vi "XY8_Pulse_Manipulation.vi"(8 "Numeric 2":i32, 9 "Invert?":bool, 10 "Numeric":i32, 11 "MW Step Size":dbl=2e-09) -> (3 "Tau":dbl)   [LabVIEW 2024]
uses:
  <vilib>/Utility/error.llb/DialogTypeEnum.ctl
  SpinCore_API_file_location.vi
panel:
  out "output array 2":T1(array[cluster])
  in  "clock_freq (MHz) 2":dbl=500.0
  out "x+y 11":dbl
  out "x+y 10":dbl
  out "x+y 9":dbl
  out "x+y 8":dbl
  out "x+y 7":dbl
  out "x+y 39":dbl
  out "x+y 38":dbl
  out "x+y 37":dbl
  out "x+y 36":dbl
  out "x+y 35":dbl
  out "x+y 34":dbl
  out "x+y 33":dbl
  out "x+y 32":dbl
  out "x+y 31":dbl
  out "x+y 30":dbl
  out "x+y 29":dbl
  out "x+y 28":dbl
  out "x+y 27":dbl
  out "x+y 26":dbl
  out "x+y 25":dbl
  out "x+y 24":dbl
  out "x+y 23":dbl
  out "x+y 22":dbl
  out "x+y 21":dbl
  out "x+y 20":dbl
  out "x+y 19":dbl
  out "x+y 18":dbl
  out "x+y 17":dbl
  out "x+y 16":dbl
  out "x+y 15":dbl
  out "x+y 14":dbl
  out "x+y 13":dbl
  out "x+y 12":dbl
  in  "# of Instructions":u32=49
  in  "Instructions":T1(array[cluster])=[{"Instruct Data"=0, "Op Code"=0, "Flags"=[FALSE, FALSE, TRUE, FALSE, FALSE, FALSE, FALSE, TRUE, FALSE, FALSE, FALSE, FALSE, FALSE, FALSE, FALSE, FALSE, FALSE, FALSE, FALSE, FALSE, FALSE, FALSE, FALSE, TRUE], "Comments"="0 Triggers", "Time (s)"=1e-07}, {"Instruct Data"=0, "Op Code"=0, "Flags"=[FALSE, FALSE, FALSE, FALSE, FALSE, FALSE, FALSE, TRUE, FALSE, FALSE, FALSE, FALSE, FALSE, FALSE, FALSE, FALSE, FALSE, FALSE, FALSE, FALSE, FALSE, FALSE, FALSE, FALSE], "Comments"="1 Dark ", "Time (s)"=0.00024}, {"Instruct Data"=0, "Op Code"=0, "Flags"=[FALSE, FALSE, FALSE, FALSE, FALSE, FALSE, FALSE, TRUE, FALSE, FALSE, FALSE, FALSE, FALSE, FALSE, FALSE, FALSE, FALSE, FALSE, FALSE, FALSE, FALSE, FALSE, FALSE, FALSE], "Comments"="2 AOM Buffer", "Time (s)"=5e-07}, {"Instruct Data"=0, "Op Code"=0, "Flags"=[TRUE, FALSE, FALSE, TRUE, FALSE, FALSE, FALSE, TRUE, FALSE, FALSE, FALSE, FALSE, FALSE, FALSE, FALSE, FALSE, FALSE, FALSE, FALSE, FALSE, FALSE, FALSE, FALSE, FALSE], "Comments"="3 pi/2", "Time (s)"=3.6e-08}, {"Instruct Data"=0, "Op Code"=0, "Flags"=[FALSE, FALSE, FALSE, FALSE, FALSE, FALSE, FALSE, TRUE, FALSE, FALSE, FALSE, FALSE, FALSE, FALSE, FALSE, FALSE, FALSE, FALSE, FALSE, FALSE, FALSE, FALSE, FALSE, FALSE], "Comments"="4 tau/2", "Time (s)"=2.313e-05}, {"Instruct Data"=0, "Op Code"=0, "Flags"=[TRUE, FALSE, FALSE, TRUE, FALSE, FALSE, FALSE, TRUE, FALSE, FALSE, FALSE, FALSE, FALSE, FALSE, FALSE, FALSE, FALSE, FALSE, FALSE, FALSE, FALSE, FALSE, FALSE, FALSE], "Comments"="5  Pi_X", "Time (s)"=6.7e-08}, {"Instruct Data"=0, "Op Code"=0, "Flags"=[FALSE, FALSE, FALSE, FALSE, FALSE, FALSE, FALSE, TRUE, FALSE, FALSE, FALSE, FALSE, FALSE, FALSE, FALSE, FALSE, FALSE, FALSE, FALSE, FALSE, FALSE, FALSE, FALSE, FALSE], "Comments"="6 Tau", "Time (s)"=4.626e-05}, {"Instruct Data"=0, "Op Code"=0, "Flags"=[TRUE, FALSE, FALSE, FALSE, TRUE, FALSE, FALSE, TRUE, FALSE, FALSE, FALSE, FALSE, FALSE, FALSE, FALSE, FALSE, FALSE, FALSE, FALSE, FALSE, FALSE, FALSE, FALSE, FALSE], "Comments"="7 Pi_Y", "Time (s)"=7e-08}, {"Instruct Data"=0, "Op Code"=0, "Flags"=[FALSE, FALSE, FALSE, FALSE, FALSE, FALSE, FALSE, TRUE, FALSE, FALSE, FALSE, FALSE, FALSE, FALSE, FALSE, FALSE, FALSE, FALSE, FALSE, FALSE, FALSE, FALSE, FALSE, FALSE], "Comments"="8 Tau", "Time (s)"=4.626e-05}, {"Instruct Data"=0, "Op Code"=0, "Flags"=[TRUE, FALSE, FALSE, TRUE, FALSE, FALSE, FALSE, TRUE, FALSE, FALSE, FALSE, FALSE, FALSE, FALSE, FALSE, FALSE, FALSE, FALSE, FALSE, FALSE, FALSE, FALSE, FALSE, FALSE], "Comments"="9 Pi_X", "Time (s)"=6.7e-08}, {"Instruct Data"=0, "Op Code"=0, "Flags"=[FALSE, FALSE, FALSE, FALSE, FALSE, FALSE, FALSE, TRUE, FALSE, FALSE, FALSE, FALSE, FALSE, FALSE, FALSE, FALSE, FALSE, FALSE, FALSE, FALSE, FALSE, FALSE, FALSE, FALSE], "Comments"="10 tau", "Time (s)"=4.626e-05}, {"Instruct Data"=0, "Op Code"=0, "Flags"=[TRUE, FALSE, FALSE, FALSE, TRUE, FALSE, FALSE, TRUE, FALSE, FALSE, FALSE, FALSE, FALSE, FALSE, FALSE, FALSE, FALSE, FALSE, FALSE, FALSE, FALSE, FALSE, FALSE, FALSE], "Comments"="11 Pi_Y", "Time (s)"=7e-08}, {"Instruct Data"=0, "Op Code"=0, "Flags"=[FALSE, FALSE, FALSE, FALSE, FALSE, FALSE, FALSE, TRUE, FALSE, FALSE, FALSE, FALSE, FALSE, FALSE, FALSE, FALSE, FALSE, FALSE, FALSE, FALSE, FALSE, FALSE, FALSE, FALSE], "Comments"="12 Tau", "Time (s)"=4.626e-05}, {"Instruct Data"=0, "Op Code"=0, "Flags"=[TRUE, FALSE, FALSE, FALSE, TRUE, FALSE, FALSE, TRUE, FALSE, FALSE, FALSE, FALSE, FALSE, FALSE, FALSE, FALSE, FALSE, FALSE, FALSE, FALSE, FALSE, FALSE, FALSE, FALSE], "Comments"="13 Pi_Y", "Time (s)"=7e-08}, {"Instruct Data"=0, "Op Code"=0, "Flags"=[FALSE, FALSE, FALSE, FALSE, FALSE, FALSE, FALSE, TRUE, FALSE, FALSE, FALSE, FALSE, FALSE, FALSE, FALSE, FALSE, FALSE, FALSE, FALSE, FALSE, FALSE, FALSE, FALSE, FALSE], "Comments"="14 tau", "Time (s)"=4.626e-05}, {"Instruct Data"=0, "Op Code"=0, "Flags"=[TRUE, FALSE, FALSE, TRUE, FALSE, FALSE, FALSE, TRUE, FALSE, FALSE, FALSE, FALSE, FALSE, FALSE, FALSE, FALSE, FALSE, FALSE, FALSE, FALSE, FALSE, FALSE, FALSE, FALSE], "Comments"="15 Pi_X", "Time (s)"=6.7e-08}, {"Instruct Data"=0, "Op Code"=0, "Flags"=[FALSE, FALSE, FALSE, FALSE, FALSE, FALSE, FALSE, TRUE, FALSE, FALSE, FALSE, FALSE, FALSE, FALSE, FALSE, FALSE, FALSE, FALSE, FALSE, FALSE, FALSE, FALSE, FALSE, FALSE], "Comments"="16  tau", "Time (s)"=4.626e-05}, {"Instruct Data"=0, "Op Code"=0, "Flags"=[TRUE, FALSE, FALSE, FALSE, TRUE, FALSE, FALSE, TRUE, FALSE, FALSE, FALSE, FALSE, FALSE, FALSE, FALSE, FALSE, FALSE, FALSE, FALSE, FALSE, FALSE, FALSE, FALSE, FALSE], "Comments"="17 Pi_Y", "Time (s)"=7e-08}, {"Instruct Data"=0, "Op Code"=0, "Flags"=[FALSE, FALSE, FALSE, FALSE, FALSE, FALSE, FALSE, TRUE, FALSE, FALSE, FALSE, FALSE, FALSE, FALSE, FALSE, FALSE, FALSE, FALSE, FALSE, FALSE, FALSE, FALSE, FALSE, FALSE], "Comments"="18 tau", "Time (s)"=4.626e-05}, {"Instruct Data"=0, "Op Code"=0, "Flags"=[TRUE, FALSE, FALSE, TRUE, FALSE, FALSE, FALSE, TRUE, FALSE, FALSE, FALSE, FALSE, FALSE, FALSE, FALSE, FALSE, FALSE, FALSE, FALSE, FALSE, FALSE, FALSE, FALSE, FALSE], "Comments"="19 pi_X", "Time (s)"=6.7e-08}, {"Instruct Data"=0, "Op Code"=0, "Flags"=[FALSE, FALSE, FALSE, FALSE, FALSE, FALSE, FALSE, TRUE, FALSE, FALSE, FALSE, FALSE, FALSE, FALSE, FALSE, FALSE, FALSE, FALSE, FALSE, FALSE, FALSE, FALSE, FALSE, FALSE], "Comments"="20  tau/2", "Time (s)"=2.313e-05}, {"Instruct Data"=0, "Op Code"=0, "Flags"=[TRUE, FALSE, FALSE, TRUE, FALSE, FALSE, FALSE, TRUE, FALSE, FALSE, FALSE, FALSE, FALSE, FALSE, FALSE, FALSE, FALSE, FALSE, FALSE, FALSE, FALSE, FALSE, FALSE, FALSE], "Comments"="21 pi/2", "Time (s)"=3.6e-08}, {"Instruct Data"=0, "Op Code"=0, "Flags"=[FALSE, TRUE, FALSE, FALSE, FALSE, FALSE, FALSE, TRUE, FALSE, FALSE, FALSE, FALSE, FALSE, FALSE, FALSE, FALSE, FALSE, FALSE, FALSE, FALSE, FALSE, FALSE, FALSE, FALSE], "Comments"="22 AOM Buffer", "Time (s)"=5e-07}, {"Instruct Data"=0, "Op Code"=0, "Flags"=[FALSE, TRUE, FALSE, FALSE, FALSE, FALSE, FALSE, FALSE, FALSE, FALSE, FALSE, FALSE, FALSE, FALSE, FALSE, FALSE, FALSE, FALSE, FALSE, FALSE, FALSE, FALSE, FALSE, FALSE], "Comments"="23  Inhibit off", "Time (s)"=5e-07}, {"Instruct Data"=0, "Op Code"=0, "Flags"=[FALSE, TRUE, FALSE, FALSE, FALSE, FALSE, FALSE, TRUE, FALSE, FALSE, FALSE, FALSE, FALSE, FALSE, FALSE, FALSE, FALSE, FALSE, FALSE, FALSE, FALSE, FALSE, FALSE, FALSE], "Comments"="24  AOM", "Time (s)"=5e-06}, {"Instruct Data"=0, "Op Code"=0, "Flags"=[FALSE, FALSE, FALSE, FALSE, FALSE, FALSE, FALSE, TRUE, FALSE, FALSE, FALSE, FALSE, FALSE, FALSE, FALSE, FALSE, FALSE, FALSE, FALSE, FALSE, FALSE, FALSE, FALSE, FALSE], "Comments"="25  Dark", "Time (s)"=0.00024}, {"Instruct Data"=0, "Op Code"=0, "Flags"=[FALSE, FALSE, FALSE, FALSE, FALSE, FALSE, FALSE, TRUE, FALSE, FALSE, FALSE, FALSE, FALSE, FALSE, FALSE, FALSE, FALSE, FALSE, FALSE, FALSE, FALSE, FALSE, FALSE, FALSE], "Comments"="26  AOm buffer", "Time (s)"=5e-07}, {"Instruct Data"=0, "Op Code"=0, "Flags"=[TRUE, FALSE, FALSE, TRUE, FALSE, FALSE, FALSE, TRUE, FALSE, FALSE, FALSE, FALSE, FALSE, FALSE, FALSE, FALSE, FALSE, FALSE, FALSE, FALSE, FALSE, FALSE, FALSE, FALSE], "Comments"="27  pi/2", "Time (s)"=3.6e-08}, {"Instruct Data"=0, "Op Code"=0, "Flags"=[FALSE, FALSE, FALSE, FALSE, FALSE, FALSE, FALSE, TRUE, FALSE, FALSE, FALSE, FALSE, FALSE, FALSE, FALSE, FALSE, FALSE, FALSE, FALSE, FALSE, FALSE, FALSE, FALSE, FALSE], "Comments"="28  tau/2", "Time (s)"=2.313e-05}, {"Instruct Data"=0, "Op Code"=0, "Flags"=[TRUE, FALSE, FALSE, TRUE, FALSE, FALSE, FALSE, TRUE, FALSE, FALSE, FALSE, FALSE, FALSE, FALSE, FALSE, FALSE, FALSE, FALSE, FALSE, FALSE, FALSE, FALSE, FALSE, FALSE], "Comments"="29  pi_X", "Time (s)"=6.7e-08}, {"Instruct Data"=0, "Op Code"=0, "Flags"=[FALSE, FALSE, FALSE, FALSE, FALSE, FALSE, FALSE, TRUE, FALSE, FALSE, FALSE, FALSE, FALSE, FALSE, FALSE, FALSE, FALSE, FALSE, FALSE, FALSE, FALSE, FALSE, FALSE, FALSE], "Comments"="30  tau", "Time (s)"=4.626e-05}, {"Instruct Data"=0, "Op Code"=0, "Flags"=[TRUE, FALSE, FALSE, FALSE, TRUE, FALSE, FALSE, TRUE, FALSE, FALSE, FALSE, FALSE, FALSE, FALSE, FALSE, FALSE, FALSE, FALSE, FALSE, FALSE, FALSE, FALSE, FALSE, FALSE], "Comments"="31  Pi_y", "Time (s)"=7e-08}, {"Instruct Data"=0, "Op Code"=0, "Flags"=[FALSE, FALSE, FALSE, FALSE, FALSE, FALSE, FALSE, TRUE, FALSE, FALSE, FALSE, FALSE, FALSE, FALSE, FALSE, FALSE, FALSE, FALSE, FALSE, FALSE, FALSE, FALSE, FALSE, FALSE], "Comments"="32  tau", "Time (s)"=4.626e-05}, {"Instruct Data"=0, "Op Code"=0, "Flags"=[TRUE, FALSE, FALSE, TRUE, FALSE, FALSE, FALSE, TRUE, FALSE, FALSE, FALSE, FALSE, FALSE, FALSE, FALSE, FALSE, FALSE, FALSE, FALSE, FALSE, FALSE, FALSE, FALSE, FALSE], "Comments"="33  Pi_X", "Time (s)"=6.7e-08}, {"Instruct Data"=0, "Op Code"=0, "Flags"=[FALSE, FALSE, FALSE, FALSE, FALSE, FALSE, FALSE, TRUE, FALSE, FALSE, FALSE, FALSE, FALSE, FALSE, FALSE, FALSE, FALSE, FALSE, FALSE, FALSE, FALSE, FALSE, FALSE, FALSE], "Comments"="34  tau", "Time (s)"=4.626e-05}, {"Instruct Data"=0, "Op Code"=0, "Flags"=[TRUE, FALSE, FALSE, FALSE, TRUE, FALSE, FALSE, TRUE, FALSE, FALSE, FALSE, FALSE, FALSE, FALSE, FALSE, FALSE, FALSE, FALSE, FALSE, FALSE, FALSE, FALSE, FALSE, FALSE], "Comments"="35 Pi_Y", "Time (s)"=7e-08}, {"Instruct Data"=0, "Op Code"=0, "Flags"=[FALSE, FALSE, FALSE, FALSE, FALSE, FALSE, FALSE, TRUE, FALSE, FALSE, FALSE, FALSE, FALSE, FALSE, FALSE, FALSE, FALSE, FALSE, FALSE, FALSE, FALSE, FALSE, FALSE, FALSE], "Comments"="36  tau", "Time (s)"=4.626e-05}, {"Instruct Data"=0, "Op Code"=0, "Flags"=[TRUE, FALSE, FALSE, FALSE, TRUE, FALSE, FALSE, TRUE, FALSE, FALSE, FALSE, FALSE, FALSE, FALSE, FALSE, FALSE, FALSE, FALSE, FALSE, FALSE, FALSE, FALSE, FALSE, FALSE], "Comments"="37  Pi_Y", "Time (s)"=7e-08}, {"Instruct Data"=0, "Op Code"=0, "Flags"=[FALSE, FALSE, FALSE, FALSE, FALSE, FALSE, FALSE, TRUE, FALSE, FALSE, FALSE, FALSE, FALSE, FALSE, FALSE, FALSE, FALSE, FALSE, FALSE, FALSE, FALSE, FALSE, FALSE, FALSE], "Comments"="38  tau", "Time (s)"=4.626e-05}, {"Instruct Data"=0, "Op Code"=0, "Flags"=[TRUE, FALSE, FALSE, TRUE, FALSE, FALSE, FALSE, TRUE, FALSE, FALSE, FALSE, FALSE, FALSE, FALSE, FALSE, FALSE, FALSE, FALSE, FALSE, FALSE, FALSE, FALSE, FALSE, FALSE], "Comments"="39  Pi_X", "Time (s)"=6.7e-08}, {"Instruct Data"=0, "Op Code"=0, "Flags"=[FALSE, FALSE, FALSE, FALSE, FALSE, FALSE, FALSE, TRUE, FALSE, FALSE, FALSE, FALSE, FALSE, FALSE, FALSE, FALSE, FALSE, FALSE, FALSE, FALSE, FALSE, FALSE, FALSE, FALSE], "Comments"="40  tau", "Time (s)"=4.626e-05}, {"Instruct Data"=0, "Op Code"=0, "Flags"=[TRUE, FALSE, FALSE, FALSE, TRUE, FALSE, FALSE, TRUE, FALSE, FALSE, FALSE, FALSE, FALSE, FALSE, FALSE, FALSE, FALSE, FALSE, FALSE, FALSE, FALSE, FALSE, FALSE, FALSE], "Comments"="41  pi_Y", "Time (s)"=7e-08}, {"Instruct Data"=0, "Op Code"=0, "Flags"=[FALSE, FALSE, FALSE, FALSE, FALSE, FALSE, FALSE, TRUE, FALSE, FALSE, FALSE, FALSE, FALSE, FALSE, FALSE, FALSE, FALSE, FALSE, FALSE, FALSE, FALSE, FALSE, FALSE, FALSE], "Comments"="42  tau", "Time (s)"=4.626e-05}, {"Instruct Data"=0, "Op Code"=0, "Flags"=[TRUE, FALSE, FALSE, TRUE, FALSE, FALSE, FALSE, TRUE, FALSE, FALSE, FALSE, FALSE, FALSE, FALSE, FALSE, FALSE, FALSE, FALSE, FALSE, FALSE, FALSE, FALSE, FALSE, FALSE], "Comments"="43  Pi_x", "Time (s)"=6.7e-08}, {"Instruct Data"=0, "Op Code"=0, "Flags"=[FALSE, FALSE, FALSE, FALSE, FALSE, FALSE, FALSE, TRUE, FALSE, FALSE, FALSE, FALSE, FALSE, FALSE, FALSE, FALSE, FALSE, FALSE, FALSE, FALSE, FALSE, FALSE, FALSE, FALSE], "Comments"="44  tau/2", "Time (s)"=2.313e-05}, {"Instruct Data"=0, "Op Code"=0, "Flags"=[TRUE, FALSE, FALSE, TRUE, FALSE, FALSE, FALSE, TRUE, FALSE, FALSE, FALSE, FALSE, FALSE, FALSE, FALSE, FALSE, FALSE, FALSE, FALSE, FALSE, FALSE, FALSE, FALSE, FALSE], "Comments"="45  3Pi/2", "Time (s)"=1.01e-07}, {"Instruct Data"=0, "Op Code"=0, "Flags"=[FALSE, TRUE, FALSE, FALSE, FALSE, FALSE, FALSE, TRUE, FALSE, FALSE, FALSE, FALSE, FALSE, FALSE, FALSE, FALSE, FALSE, FALSE, FALSE, FALSE, FALSE, FALSE, FALSE, FALSE], "Comments"="46  AOM Buffer", "Time (s)"=5e-07}, {"Instruct Data"=0, "Op Code"=0, "Flags"=[FALSE, TRUE, FALSE, FALSE, FALSE, FALSE, FALSE, FALSE, FALSE, FALSE, FALSE, FALSE, FALSE, FALSE, FALSE, FALSE, FALSE, FALSE, FALSE, FALSE, FALSE, FALSE, FALSE, FALSE], "Comments"="47  Inhibit off", "Time (s)"=5e-07}, {"Instruct Data"=0, "Op Code"=6, "Flags"=[FALSE, TRUE, FALSE, FALSE, FALSE, FALSE, FALSE, TRUE, FALSE, FALSE, FALSE, FALSE, FALSE, FALSE, FALSE, FALSE, FALSE, FALSE, FALSE, FALSE, FALSE, FALSE, FALSE, FALSE], "Comments"="48  AOM", "Time (s)"=5e-06}] {"Time (s)" format="%.3p"; "Op Code" items=["Continue", "Stop", "Loop", "End Loop", "JSR", "RTS", "Branch", "Long Delay", "Wait"]}
  out "output array":T1(array[cluster])
  in  "clock_freq (MHz)":dbl=500.0
  out "x+y 2":dbl
  out "x+y 3":dbl
  out "x+y 4":dbl
  out "x+y 5":dbl
  out "x+y 6":dbl
  # "1"
  # "2"
  # "3"
  # "4"
  # "5"
  # "6"
  # "7"
  # "8"
  # "9"
  # "10"
  # "11"
  # "12"
  # "13"
  # "14"
  # "15"
  # "16"
  # "17"
  # "18"
  # "19"
  # "20"
  # "21"
  # "22"
  # "23"
  # "24"
types:
  T1 = cluster{"Instruct Data":i32, "Op Code":i32, "Flags":bool[], "Comments":string, "Time (s)":dbl}[]
  T2 = typedef "DialogTypeEnum.ctl" = enum16{"no dialog", "OK message", "continue or stop message", "auto error handling dialog", "OK message + warnings", "continue/stop + warnings"}
  T3 = enum16{"Pulse Program", "Frequency Registers", "TX Phase Registers", "RX Phase Registers"}
  T4 = cluster{"Instruct Data":i32, "Op Code":i32, "Flags":bool[], "Comments":string, "Time (s)":dbl}
  T5 = cluster{"Instruct Data":i32, "Op Code":i32, "Flags":bool[], "Comments":string, dbl}
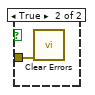
[diagram p2: hidden frame]
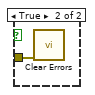
[diagram p4: hidden frame]
diagram:
  n1 = case shown="False" "Invert?" {
    tunnel: "Instructions" -> [w6 w361]
    tunnel: "# of Instructions" -> [w8 w360]
    tunnel: "# of Instructions" -> [w7 w359]
    tunnel: "MW Step Size" -> [w10 w358]
    tunnel: [w9 w357] -> w1
    frame False {
      n2 = flat-sequence {
        tunnel: w8 -> [w194]
        tunnel: [w12] -> _
        tunnel: w10 -> [w193]
        tunnel: [w13] -> w9
        tunnel: w7 -> [w12]
        tunnel: w6 -> [w11]
        frame #0 {
          # "tau"
          # "tau"
          # "tau"
          # "tau"
          # "tau"
          # "tau"
          # "tau/2"
          # "DARK"
          n3 = Reshape Array "Reshape Array"(w11, w194) -> (w269:T1)
          n4 = Wait (ms)(milliseconds to wait=u32 10) -> ()  [unwired: 1 out]
          n5 = Index Array "Index Array"(array=w269, index=6) -> (element=w268:T4)
          n6 = for {
            N: "Numeric 2" -> [_]
            tunnel: [w348] -> w265
            tunnel: [w347] -> w27 mode=indexing
            tunnel: w193 -> [w347]
            i -> [w349]
            n7 = Multiply(x=w347, y=w349) -> (x*y=w348:dbl)
          }
          n8 = Unbundle By Name "Unbundle By Name"(w268) -> ("Instruct Data"=w274:i32, "Op Code"=w273:i32, "Flags"=w272:bool[], "Comments"=w271:string, "Time (s)"=w270:dbl)
          n9 = Add(x=w270, y=w265) -> (x+y=w13:dbl)
          n10 = for {
            N: "Numeric 2" -> [_]
            tunnel: [w345] -> w248
            tunnel: w27 -> [w344] mode=indexing
            i -> [w346]
            n11 = Multiply(x=w344, y=w346) -> (x*y=w345:dbl)
          }
          n12 = for {
            N: "Numeric 2" -> [_]
            tunnel: [w342] -> w236
            tunnel: w27 -> [w341] mode=indexing
            i -> [w343]
            n13 = Multiply(x=w341, y=w343) -> (x*y=w342:dbl)
          }
          n14 = for {
            N: "Numeric 2" -> [_]
            tunnel: [w339] -> w225
            tunnel: w27 -> [w338] mode=indexing
            i -> [w340]
            n15 = Multiply(x=w338, y=w340) -> (x*y=w339:dbl)
          }
          n16 = for {
            N: "Numeric 2" -> [_]
            tunnel: [w330] -> w183
            tunnel: w27 -> [w329] mode=indexing
            i -> [w331]
            n17 = Multiply(x=w329, y=w331) -> (x*y=w330:dbl)
          }
          n18 = for {
            N: "Numeric 2" -> [_]
            tunnel: [w327] -> w171
            tunnel: w27 -> [w326] mode=indexing
            i -> [w328]
            n19 = Multiply(x=w326, y=w328) -> (x*y=w327:dbl)
          }
          n20 = for {
            N: "Numeric 2" -> [_]
            tunnel: [w324] -> w159
            tunnel: w27 -> [w323] mode=indexing
            i -> [w325]
            n21 = Multiply(x=w323, y=w325) -> (x*y=w324:dbl)
          }
          n22 = for {
            N: "Numeric 2" -> [_]
            tunnel: [w321] -> w147
            tunnel: w27 -> [w320] mode=indexing
            i -> [w322]
            n23 = Multiply(x=w320, y=w322) -> (x*y=w321:dbl)
          }
          n24 = for {
            N: "Numeric 2" -> [_]
            tunnel: [w318] -> w135
            tunnel: w27 -> [w317] mode=indexing
            i -> [w319]
            n25 = Multiply(x=w317, y=w319) -> (x*y=w318:dbl)
          }
          n26 = Bundle("Instruct Data"=w274, "Op Code"=w273, "Flags"=w272, "Comments"=w271, w13) -> (w266:T5)  [unwired: 1 in]
          n27 = Replace Array Subset "Replace Array Subset"(array=w269, new element=w266, index=6) -> (w247:T1)
          n28 = Index Array "Index Array"(array=w247, index=8) -> (element=w251:T4)
          n29 = Unbundle(w251) -> ("Instruct Data"=w257:i32, "Op Code"=w256:i32, "Flags"=w255:bool[], "Comments"=w254:string, "Time (s)"=w253:dbl)
          n30 = Add(x=w253, y=w248) -> (x+y=w252:dbl)
          "x+y 11" <- w252
          n31 = Bundle("Instruct Data"=w257, "Op Code"=w256, "Flags"=w255, "Comments"=w254, w252) -> (w249:T5)  [unwired: 1 in]
          n32 = Replace Array Subset "Replace Array Subset"(array=w247, new element=w249, index=8) -> (w235:T1)
          n33 = Index Array "Index Array"(array=w235, index=10) -> (element=w239:T4)
          n34 = Unbundle(w239) -> ("Instruct Data"=w245:i32, "Op Code"=w244:i32, "Flags"=w243:bool[], "Comments"=w242:string, "Time (s)"=w241:dbl)
          n35 = Add(x=w241, y=w236) -> (x+y=w240:dbl)
          "x+y 10" <- w240
          n36 = Bundle("Instruct Data"=w245, "Op Code"=w244, "Flags"=w243, "Comments"=w242, w240) -> (w237:T5)  [unwired: 1 in]
          n37 = Replace Array Subset "Replace Array Subset"(array=w235, new element=w237, index=10) -> (w224:T1)
          n38 = Index Array "Index Array"(array=w224, index=12) -> (element=w228:T4)
          n39 = Unbundle(w228) -> ("Instruct Data"=w234:i32, "Op Code"=w233:i32, "Flags"=w232:bool[], "Comments"=w231:string, "Time (s)"=w230:dbl)
          n40 = Add(x=w230, y=w225) -> (x+y=w229:dbl)
          "x+y 9" <- w229
          n41 = Bundle("Instruct Data"=w234, "Op Code"=w233, "Flags"=w232, "Comments"=w231, w229) -> (w226:T5)  [unwired: 1 in]
          n42 = Replace Array Subset "Replace Array Subset"(array=w224, new element=w226, index=12) -> (w181:T1)
          n43 = Index Array "Index Array"(array=w181, index=14) -> (element=w186:T4)
          n44 = Unbundle(w186) -> ("Instruct Data"=w192:i32, "Op Code"=w191:i32, "Flags"=w190:bool[], "Comments"=w189:string, "Time (s)"=w188:dbl)
          n45 = Add(x=w188, y=w183) -> (x+y=w187:dbl)
          "x+y 39" <- w187
          n46 = Bundle("Instruct Data"=w192, "Op Code"=w191, "Flags"=w190, "Comments"=w189, w187) -> (w184:T5)  [unwired: 1 in]
          n47 = Replace Array Subset "Replace Array Subset"(array=w181, new element=w184, index=14) -> (w169:T1)
          n48 = Index Array "Index Array"(array=w169, index=16) -> (element=w174:T4)
          n49 = Unbundle(w174) -> ("Instruct Data"=w180:i32, "Op Code"=w179:i32, "Flags"=w178:bool[], "Comments"=w177:string, "Time (s)"=w176:dbl)
          n50 = Add(x=w176, y=w171) -> (x+y=w175:dbl)
          "x+y 38" <- w175
          n51 = Bundle("Instruct Data"=w180, "Op Code"=w179, "Flags"=w178, "Comments"=w177, w175) -> (w172:T5)  [unwired: 1 in]
          n52 = Replace Array Subset "Replace Array Subset"(array=w169, new element=w172, index=16) -> (w157:T1)
          n53 = for {
            N: "Numeric 2" -> [_]
            tunnel: [w315] -> w124
            tunnel: w27 -> [w314] mode=indexing
            i -> [w316]
            n54 = Multiply(x=w314, y=w316) -> (x*y=w315:dbl)
          }
          n55 = for {
            N: "Numeric 2" -> [_]
            tunnel: [w312] -> w113
            tunnel: w27 -> [w311] mode=indexing
            i -> [w313]
            n56 = Multiply(x=w311, y=w313) -> (x*y=w312:dbl)
          }
          n57 = for {
            N: "Numeric 2" -> [_]
            tunnel: [w309] -> w102
            tunnel: w27 -> [w308] mode=indexing
            i -> [w310]
            n58 = Multiply(x=w308, y=w310) -> (x*y=w309:dbl)
          }
          n59 = for {
            N: "Numeric 2" -> [_]
            tunnel: [w303] -> w80
            tunnel: w27 -> [w302] mode=indexing
            i -> [w304]
            n60 = Multiply(x=w302, y=w304) -> (x*y=w303:dbl)
          }
          n61 = for {
            N: "Numeric 2" -> [_]
            tunnel: [w306] -> w91
            tunnel: w27 -> [w305] mode=indexing
            i -> [w307]
            n62 = Multiply(x=w305, y=w307) -> (x*y=w306:dbl)
          }
          n63 = for {
            N: "Numeric 2" -> [_]
            tunnel: [w297] -> w25
            tunnel: w27 -> [w296] mode=indexing
            i -> [w298]
            n64 = Multiply(x=w296, y=w298) -> (x*y=w297:dbl)
          }
          n65 = for {
            N: "Numeric 2" -> [_]
            tunnel: [w300] -> w16
            tunnel: w27 -> [w299] mode=indexing
            i -> [w301]
            n66 = Multiply(x=w299, y=w301) -> (x*y=w300:dbl)
          }
          n67 = for {
            N: "Numeric 2" -> [_]
            tunnel: [w291] -> w19
            tunnel: w27 -> [w290] mode=indexing
            i -> [w292]
            n68 = Multiply(x=w290, y=w292) -> (x*y=w291:dbl)
          }
          n69 = for {
            N: "Numeric 2" -> [_]
            tunnel: [w294] -> w22
            tunnel: w27 -> [w293] mode=indexing
            i -> [w295]
            n70 = Multiply(x=w293, y=w295) -> (x*y=w294:dbl)
          }
          n71 = for {
            N: "Numeric 2" -> [_]
            tunnel: [w336] -> w212
            tunnel: [w335] -> _ mode=indexing
            tunnel: w27 -> [w335] mode=indexing
            i -> [w337]
            n72 = Multiply(x=w335, y=w337) -> (x*y=w336:dbl)
          }
          n73 = for {
            N: "Numeric 2" -> [_]
            tunnel: [w333] -> w199
            tunnel: [w332] -> _ mode=indexing
            tunnel: w27 -> [w332] mode=indexing
            i -> [w334]
            n74 = Multiply(x=w332, y=w334) -> (x*y=w333:dbl)
          }
          n75 = Index Array "Index Array"(array=w157, index=18) -> (element=w162:T4)
          n76 = Unbundle(w162) -> ("Instruct Data"=w168:i32, "Op Code"=w167:i32, "Flags"=w166:bool[], "Comments"=w165:string, "Time (s)"=w164:dbl)
          n77 = Add(x=w164, y=w159) -> (x+y=w163:dbl)
          "x+y 37" <- w163
          n78 = Bundle("Instruct Data"=w168, "Op Code"=w167, "Flags"=w166, "Comments"=w165, w163) -> (w160:T5)  [unwired: 1 in]
          n79 = Multiply(x=8.0, y=w199) -> (x*y=w197:dbl)
          n80 = Replace Array Subset "Replace Array Subset"(array=w157, new element=w160, index=18) -> (w145:T1)
          n81 = Multiply(x=8.0, y=w212) -> (x*y=w210:dbl)
          n82 = Index Array "Index Array"(array=w145, index=30) -> (element=w150:T4)
          n83 = Unbundle(w150) -> ("Instruct Data"=w156:i32, "Op Code"=w155:i32, "Flags"=w154:bool[], "Comments"=w153:string, "Time (s)"=w152:dbl)
          n84 = Add(x=w152, y=w147) -> (x+y=w151:dbl)
          "x+y 36" <- w151
          n85 = Bundle("Instruct Data"=w156, "Op Code"=w155, "Flags"=w154, "Comments"=w153, w151) -> (w148:T5)  [unwired: 1 in]
          n86 = Divide(x=w22, y=2.0) -> (x/y=w21:sgl)
          n87 = Replace Array Subset "Replace Array Subset"(array=w145, new element=w148, index=30) -> (w38:T1)
          n88 = Divide(x=w19, y=2.0) -> (x/y=w18:sgl)
          n89 = Index Array "Index Array"(array=w38, index=32) -> (element=w138:T4)
          n90 = Unbundle(w138) -> ("Instruct Data"=w144:i32, "Op Code"=w143:i32, "Flags"=w142:bool[], "Comments"=w141:string, "Time (s)"=w140:dbl)
          n91 = Add(x=w140, y=w135) -> (x+y=w139:dbl)
          "x+y 35" <- w139
          n92 = Bundle("Instruct Data"=w144, "Op Code"=w143, "Flags"=w142, "Comments"=w141, w139) -> (w136:T5)  [unwired: 1 in]
          n93 = Divide(x=w16, y=2.0) -> (x/y=w15:sgl)
          n94 = Replace Array Subset "Replace Array Subset"(array=w38, new element=w136, index=32) -> (w37:T1)
          n95 = Divide(x=w25, y=2.0) -> (x/y=w24:dbl)
          n96 = Index Array "Index Array"(array=w37, index=34) -> (element=w127:T4)
          n97 = Unbundle(w127) -> ("Instruct Data"=w133:i32, "Op Code"=w132:i32, "Flags"=w131:bool[], "Comments"=w130:string, "Time (s)"=w129:dbl)
          n98 = Add(x=w129, y=w124) -> (x+y=w128:dbl)
          "x+y 34" <- w128
          n99 = Bundle("Instruct Data"=w133, "Op Code"=w132, "Flags"=w131, "Comments"=w130, w128) -> (w125:T5)  [unwired: 1 in]
          n100 = Replace Array Subset "Replace Array Subset"(array=w37, new element=w125, index=34) -> (w36:T1)
          n101 = Index Array "Index Array"(array=w36, index=36) -> (element=w116:T4)
          n102 = Unbundle(w116) -> ("Instruct Data"=w122:i32, "Op Code"=w121:i32, "Flags"=w120:bool[], "Comments"=w119:string, "Time (s)"=w118:dbl)
          n103 = Add(x=w118, y=w113) -> (x+y=w117:dbl)
          "x+y 33" <- w117
          n104 = Bundle("Instruct Data"=w122, "Op Code"=w121, "Flags"=w120, "Comments"=w119, w117) -> (w114:T5)  [unwired: 1 in]
          n105 = Replace Array Subset "Replace Array Subset"(array=w36, new element=w114, index=36) -> (w35:T1)
          n106 = Index Array "Index Array"(array=w35, index=38) -> (element=w105:T4)
          n107 = Unbundle(w105) -> ("Instruct Data"=w111:i32, "Op Code"=w110:i32, "Flags"=w109:bool[], "Comments"=w108:string, "Time (s)"=w107:dbl)
          n108 = Add(x=w107, y=w102) -> (x+y=w106:dbl)
          "x+y 32" <- w106
          n109 = Bundle("Instruct Data"=w111, "Op Code"=w110, "Flags"=w109, "Comments"=w108, w106) -> (w103:T5)  [unwired: 1 in]
          n110 = Replace Array Subset "Replace Array Subset"(array=w35, new element=w103, index=38) -> (w34:T1)
          n111 = Index Array "Index Array"(array=w34, index=40) -> (element=w83:T4)
          n112 = Unbundle(w83) -> ("Instruct Data"=w89:i32, "Op Code"=w88:i32, "Flags"=w87:bool[], "Comments"=w86:string, "Time (s)"=w85:dbl)
          n113 = Add(x=w85, y=w80) -> (x+y=w84:dbl)
          "x+y 30" <- w84
          n114 = Bundle("Instruct Data"=w89, "Op Code"=w88, "Flags"=w87, "Comments"=w86, w84) -> (w81:T5)  [unwired: 1 in]
          n115 = Replace Array Subset "Replace Array Subset"(array=w34, new element=w81, index=40) -> (w33:T1)
          n116 = Index Array "Index Array"(array=w33, index=42) -> (element=w94:T4)
          n117 = Unbundle(w94) -> ("Instruct Data"=w100:i32, "Op Code"=w99:i32, "Flags"=w98:bool[], "Comments"=w97:string, "Time (s)"=w96:dbl)
          n118 = Add(x=w96, y=w91) -> (x+y=w95:dbl)
          "x+y 31" <- w95
          n119 = Bundle("Instruct Data"=w100, "Op Code"=w99, "Flags"=w98, "Comments"=w97, w95) -> (w92:T5)  [unwired: 1 in]
          n120 = Replace Array Subset "Replace Array Subset"(array=w33, new element=w92, index=42) -> (w32:T1)
          n121 = Index Array "Index Array"(array=w32, index=4) -> (element=w62:T4)
          n122 = Unbundle(w62) -> ("Instruct Data"=w68:i32, "Op Code"=w67:i32, "Flags"=w66:bool[], "Comments"=w65:string, "Time (s)"=w64:dbl)
          n123 = Add(x=w64, y=w24) -> (x+y=w63:dbl)
          "x+y 28" <- w63
          n124 = Bundle("Instruct Data"=w68, "Op Code"=w67, "Flags"=w66, "Comments"=w65, w63) -> (w60:T5)  [unwired: 1 in]
          n125 = Replace Array Subset "Replace Array Subset"(array=w32, new element=w60, index=4) -> (w31:T1)
          n126 = Index Array "Index Array"(array=w31, index=20) -> (element=w72:T4)
          n127 = Unbundle(w72) -> ("Instruct Data"=w78:i32, "Op Code"=w77:i32, "Flags"=w76:bool[], "Comments"=w75:string, "Time (s)"=w74:dbl)
          n128 = Add(x=w74, y=w15) -> (x+y=w73:dbl)
          "x+y 29" <- w73
          n129 = Bundle("Instruct Data"=w78, "Op Code"=w77, "Flags"=w76, "Comments"=w75, w73) -> (w70:T5)  [unwired: 1 in]
          n130 = Replace Array Subset "Replace Array Subset"(array=w31, new element=w70, index=20) -> (w30:T1)
          n131 = Index Array "Index Array"(array=w30, index=28) -> (element=w42:T4)
          n132 = Unbundle(w42) -> ("Instruct Data"=w48:i32, "Op Code"=w47:i32, "Flags"=w46:bool[], "Comments"=w45:string, "Time (s)"=w44:dbl)
          n133 = Add(x=w44, y=w18) -> (x+y=w43:dbl)
          "x+y 26" <- w43
          n134 = Bundle("Instruct Data"=w48, "Op Code"=w47, "Flags"=w46, "Comments"=w45, w43) -> (w40:T5)  [unwired: 1 in]
          n135 = Replace Array Subset "Replace Array Subset"(array=w30, new element=w40, index=28) -> (w29:T1)
          n136 = Index Array "Index Array"(array=w29, index=44) -> (element=w52:T4)
          n137 = Unbundle(w52) -> ("Instruct Data"=w58:i32, "Op Code"=w57:i32, "Flags"=w56:bool[], "Comments"=w55:string, "Time (s)"=w54:dbl)
          n138 = Add(x=w54, y=w21) -> (x+y=w53:dbl)
          "x+y 27" <- w53
          n139 = Bundle("Instruct Data"=w58, "Op Code"=w57, "Flags"=w56, "Comments"=w55, w53) -> (w50:T5)  [unwired: 1 in]
          n140 = Replace Array Subset "Replace Array Subset"(array=w29, new element=w50, index=44) -> (w28:T1)
          n141 = Index Array "Index Array"(array=w28, index=1) -> (element=w215:T4)
          n142 = Unbundle(w215) -> ("Instruct Data"=w221:i32, "Op Code"=w220:i32, "Flags"=w219:bool[], "Comments"=w218:string, "Time (s)"=w217:dbl)
          n143 = Subtract(x=w217, y=w210) -> (x-y=w216:dbl)
          "x+y 8" <- w216
          n144 = Bundle("Instruct Data"=w221, "Op Code"=w220, "Flags"=w219, "Comments"=w218, w216) -> (w213:T5)  [unwired: 1 in]
          n145 = Replace Array Subset "Replace Array Subset"(array=w28, new element=w213, index=1) -> (w196:T1)
          n146 = Index Array "Index Array"(array=w196, index=25) -> (element=w202:T4)
          n147 = Unbundle(w202) -> ("Instruct Data"=w208:i32, "Op Code"=w207:i32, "Flags"=w206:bool[], "Comments"=w205:string, "Time (s)"=w204:dbl)
          n148 = Subtract(x=w204, y=w197) -> (x-y=w203:dbl)
          "x+y 7" <- w203
          n149 = property on="Instructions" class="Arr (strict)"(error in=errorcluster {"status"=FALSE, "code"=0, "source"=""} ("error in (no error)"), "Number of Columns"=w12) -> (error out=w263:errorcluster)  [unwired: 1 in, 1 out]
          n150 = Bundle("Instruct Data"=w208, "Op Code"=w207, "Flags"=w206, "Comments"=w205, w203) -> (w200:T5)  [unwired: 1 in]
          n151 = global read "SpinCore_API_file_location.vi" "Path"() -> (w264:path)
          n152 = Replace Array Subset "Replace Array Subset"(array=w196, new element=w200, index=25) -> (w195:T1)
          "output array 2" <- w195
          n153 = call "pb_init.vi"("error in (no error)"=w263, "path in"=w264) -> ("error out"=w262:errorcluster, "path out"=w261:path)  [unwired: 8 in]
          n154 = call "pb_core_clock.vi"("error in (no error)"=w262, "clock_freq (MHz)"="clock_freq (MHz) 2", "path in"=w261) -> ("error out"=w278:errorcluster, "path out"=w279:path)  [unwired: 7 in]
          n155 = call "pb_start_programming.vi"("error in (no error)"=w278, "Device"=T3."Pulse Program", "path in"=w279) -> ("error out"=w285:errorcluster, "path out"=w289:path)  [unwired: 1 in, 6 out]
          n156 = for {
            tunnel: w195 -> [w352] mode=indexing
            shift-right: [w354] -> w287
            shift-left: w289 -> [w355]
            shift-right: [w351] -> w284
            shift-left: w285 -> [w353]
            n157 = call "pb_inst_pbonly.vi"("error in (no error)"=w353, "PB Instruction"=w352, "path in"=w355) -> ("error out"=w351:errorcluster, "path out"=w354:path)  [unwired: 2 in, 5 out]
          }
          n158 = call "pb_stop_programming.vi"("error in (no error)"=w284, "path in"=w287) -> ("error out"=w283:errorcluster, "path out"=w288:path)  [unwired: 1 in, 7 out]
          n159 = call "pb_close.vi"("error in (no error)"=w283, "path in"=w288) -> ("error out"=w276:errorcluster)  [unwired: 9 out]
          n160 = call "General Error Handler MOD.vi"("type of dialog (OK msg:1)"=DialogTypeEnum."continue or stop message", "error in (no error)"=w276) -> ("STOP?"=w280:bool, "error out"=w281:errorcluster)  [unwired: 12 out]
          n161 = case shown="False" w280 {
            tunnel: w281 -> [_ w350]
            frame False {
            }
            frame True {
              n162 = call <vilib>:"Clear Errors.vi"("error in (no error)"=w350) -> ()  [unwired: 1 in, 6 out]
            }
          }
        }
        frame #1 {
          n163 = Wait (ms)(milliseconds to wait=u32 1) -> ()  [unwired: 1 out]
        }
      }
    }
    frame True {
      n164 = flat-sequence {
        tunnel: w361 -> [w545]
        tunnel: w360 -> [w544]
        tunnel: w359 -> [w543]
        tunnel: w358 -> [w542]
        tunnel: [w541] -> w357
        frame #0 {
          # "tau"
          # "tau"
          # "tau"
          # "tau"
          # "tau"
          # "tau"
          # "tau/2"
          # "DARK"
          n165 = Reshape Array "Reshape Array"(w545, w544) -> (w620:T1)
          n166 = Wait (ms)(milliseconds to wait=u32 10) -> ()  [unwired: 1 out]
          n167 = Index Array "Index Array"(array=w620, index=6) -> (element=w619:T4)
          n168 = for {
            N: "Numeric" -> [_]
            tunnel: [w699] -> w616
            tunnel: [w698] -> w375 mode=indexing
            tunnel: w542 -> [w698]
            i -> [w700]
            n169 = Multiply(x=w698, y=w700) -> (x*y=w699:dbl)
          }
          n170 = Unbundle By Name "Unbundle By Name"(w619) -> ("Instruct Data"=w625:i32, "Op Code"=w624:i32, "Flags"=w623:bool[], "Comments"=w622:string, "Time (s)"=w621:dbl)
          n171 = Add(x=w621, y=w616) -> (x+y=w541:dbl)
          n172 = for {
            N: "Numeric" -> [_]
            tunnel: [w696] -> w599
            tunnel: w375 -> [w695] mode=indexing
            i -> [w697]
            n173 = Multiply(x=w695, y=w697) -> (x*y=w696:dbl)
          }
          n174 = for {
            N: "Numeric" -> [_]
            tunnel: [w693] -> w587
            tunnel: w375 -> [w692] mode=indexing
            i -> [w694]
            n175 = Multiply(x=w692, y=w694) -> (x*y=w693:dbl)
          }
          n176 = for {
            N: "Numeric" -> [_]
            tunnel: [w690] -> w576
            tunnel: w375 -> [w689] mode=indexing
            i -> [w691]
            n177 = Multiply(x=w689, y=w691) -> (x*y=w690:dbl)
          }
          n178 = for {
            N: "Numeric" -> [_]
            tunnel: [w681] -> w531
            tunnel: w375 -> [w680] mode=indexing
            i -> [w682]
            n179 = Multiply(x=w680, y=w682) -> (x*y=w681:dbl)
          }
          n180 = for {
            N: "Numeric" -> [_]
            tunnel: [w678] -> w519
            tunnel: w375 -> [w677] mode=indexing
            i -> [w679]
            n181 = Multiply(x=w677, y=w679) -> (x*y=w678:dbl)
          }
          n182 = for {
            N: "Numeric" -> [_]
            tunnel: [w675] -> w507
            tunnel: w375 -> [w674] mode=indexing
            i -> [w676]
            n183 = Multiply(x=w674, y=w676) -> (x*y=w675:dbl)
          }
          n184 = for {
            N: "Numeric" -> [_]
            tunnel: [w672] -> w495
            tunnel: w375 -> [w671] mode=indexing
            i -> [w673]
            n185 = Multiply(x=w671, y=w673) -> (x*y=w672:dbl)
          }
          n186 = for {
            N: "Numeric" -> [_]
            tunnel: [w669] -> w483
            tunnel: w375 -> [w668] mode=indexing
            i -> [w670]
            n187 = Multiply(x=w668, y=w670) -> (x*y=w669:dbl)
          }
          n188 = Bundle("Instruct Data"=w625, "Op Code"=w624, "Flags"=w623, "Comments"=w622, w541) -> (w617:T5)  [unwired: 1 in]
          n189 = Replace Array Subset "Replace Array Subset"(array=w620, new element=w617, index=6) -> (w598:T1)
          n190 = Index Array "Index Array"(array=w598, index=8) -> (element=w602:T4)
          n191 = Unbundle By Name "Unbundle By Name"(w602) -> ("Instruct Data"=w608:i32, "Op Code"=w607:i32, "Flags"=w606:bool[], "Comments"=w605:string, "Time (s)"=w604:dbl)
          n192 = Add(x=w604, y=w599) -> (x+y=w603:dbl)
          "x+y 2" <- w603
          n193 = Bundle("Instruct Data"=w608, "Op Code"=w607, "Flags"=w606, "Comments"=w605, w603) -> (w600:T5)  [unwired: 1 in]
          n194 = Replace Array Subset "Replace Array Subset"(array=w598, new element=w600, index=8) -> (w586:T1)
          n195 = Index Array "Index Array"(array=w586, index=10) -> (element=w590:T4)
          n196 = Unbundle By Name "Unbundle By Name"(w590) -> ("Instruct Data"=w596:i32, "Op Code"=w595:i32, "Flags"=w594:bool[], "Comments"=w593:string, "Time (s)"=w592:dbl)
          n197 = Add(x=w592, y=w587) -> (x+y=w591:dbl)
          "x+y 3" <- w591
          n198 = Bundle("Instruct Data"=w596, "Op Code"=w595, "Flags"=w594, "Comments"=w593, w591) -> (w588:T5)  [unwired: 1 in]
          n199 = Replace Array Subset "Replace Array Subset"(array=w586, new element=w588, index=10) -> (w575:T1)
          n200 = Index Array "Index Array"(array=w575, index=12) -> (element=w579:T4)
          n201 = Unbundle By Name "Unbundle By Name"(w579) -> ("Instruct Data"=w585:i32, "Op Code"=w584:i32, "Flags"=w583:bool[], "Comments"=w582:string, "Time (s)"=w581:dbl)
          n202 = Add(x=w581, y=w576) -> (x+y=w580:dbl)
          "x+y 4" <- w580
          n203 = Bundle("Instruct Data"=w585, "Op Code"=w584, "Flags"=w583, "Comments"=w582, w580) -> (w577:T5)  [unwired: 1 in]
          n204 = Replace Array Subset "Replace Array Subset"(array=w575, new element=w577, index=12) -> (w529:T1)
          n205 = Index Array "Index Array"(array=w529, index=14) -> (element=w534:T4)
          n206 = Unbundle By Name "Unbundle By Name"(w534) -> ("Instruct Data"=w540:i32, "Op Code"=w539:i32, "Flags"=w538:bool[], "Comments"=w537:string, "Time (s)"=w536:dbl)
          n207 = Add(x=w536, y=w531) -> (x+y=w535:dbl)
          "x+y 12" <- w535
          n208 = Bundle("Instruct Data"=w540, "Op Code"=w539, "Flags"=w538, "Comments"=w537, w535) -> (w532:T5)  [unwired: 1 in]
          n209 = Replace Array Subset "Replace Array Subset"(array=w529, new element=w532, index=14) -> (w517:T1)
          n210 = Index Array "Index Array"(array=w517, index=16) -> (element=w522:T4)
          n211 = Unbundle By Name "Unbundle By Name"(w522) -> ("Instruct Data"=w528:i32, "Op Code"=w527:i32, "Flags"=w526:bool[], "Comments"=w525:string, "Time (s)"=w524:dbl)
          n212 = Add(x=w524, y=w519) -> (x+y=w523:dbl)
          "x+y 13" <- w523
          n213 = Bundle("Instruct Data"=w528, "Op Code"=w527, "Flags"=w526, "Comments"=w525, w523) -> (w520:T5)  [unwired: 1 in]
          n214 = Replace Array Subset "Replace Array Subset"(array=w517, new element=w520, index=16) -> (w505:T1)
          n215 = for {
            N: "Numeric" -> [_]
            tunnel: [w666] -> w472
            tunnel: w375 -> [w665] mode=indexing
            i -> [w667]
            n216 = Multiply(x=w665, y=w667) -> (x*y=w666:dbl)
          }
          n217 = for {
            N: "Numeric" -> [_]
            tunnel: [w663] -> w461
            tunnel: w375 -> [w662] mode=indexing
            i -> [w664]
            n218 = Multiply(x=w662, y=w664) -> (x*y=w663:dbl)
          }
          n219 = for {
            N: "Numeric" -> [_]
            tunnel: [w660] -> w450
            tunnel: w375 -> [w659] mode=indexing
            i -> [w661]
            n220 = Multiply(x=w659, y=w661) -> (x*y=w660:dbl)
          }
          n221 = for {
            N: "Numeric" -> [_]
            tunnel: [w654] -> w428
            tunnel: w375 -> [w653] mode=indexing
            i -> [w655]
            n222 = Multiply(x=w653, y=w655) -> (x*y=w654:dbl)
          }
          n223 = for {
            N: "Numeric" -> [_]
            tunnel: [w657] -> w439
            tunnel: w375 -> [w656] mode=indexing
            i -> [w658]
            n224 = Multiply(x=w656, y=w658) -> (x*y=w657:dbl)
          }
          n225 = for {
            N: "Numeric" -> [_]
            tunnel: [w648] -> w373
            tunnel: w375 -> [w647] mode=indexing
            i -> [w649]
            n226 = Multiply(x=w647, y=w649) -> (x*y=w648:dbl)
          }
          n227 = for {
            N: "Numeric" -> [_]
            tunnel: [w651] -> w364
            tunnel: w375 -> [w650] mode=indexing
            i -> [w652]
            n228 = Multiply(x=w650, y=w652) -> (x*y=w651:dbl)
          }
          n229 = for {
            N: "Numeric" -> [_]
            tunnel: [w642] -> w367
            tunnel: w375 -> [w641] mode=indexing
            i -> [w643]
            n230 = Multiply(x=w641, y=w643) -> (x*y=w642:dbl)
          }
          n231 = for {
            N: "Numeric" -> [_]
            tunnel: [w645] -> w370
            tunnel: w375 -> [w644] mode=indexing
            i -> [w646]
            n232 = Multiply(x=w644, y=w646) -> (x*y=w645:dbl)
          }
          n233 = for {
            N: "Numeric" -> [_]
            tunnel: [w687] -> w563
            tunnel: [w686] -> _ mode=indexing
            tunnel: w375 -> [w686] mode=indexing
            i -> [w688]
            n234 = Multiply(x=w686, y=w688) -> (x*y=w687:dbl)
          }
          n235 = for {
            N: "Numeric" -> [_]
            tunnel: [w684] -> w550
            tunnel: [w683] -> _ mode=indexing
            tunnel: w375 -> [w683] mode=indexing
            i -> [w685]
            n236 = Multiply(x=w683, y=w685) -> (x*y=w684:dbl)
          }
          n237 = Index Array "Index Array"(array=w505, index=18) -> (element=w510:T4)
          n238 = Unbundle By Name "Unbundle By Name"(w510) -> ("Instruct Data"=w516:i32, "Op Code"=w515:i32, "Flags"=w514:bool[], "Comments"=w513:string, "Time (s)"=w512:dbl)
          n239 = Add(x=w512, y=w507) -> (x+y=w511:dbl)
          "x+y 14" <- w511
          n240 = Bundle("Instruct Data"=w516, "Op Code"=w515, "Flags"=w514, "Comments"=w513, w511) -> (w508:T5)  [unwired: 1 in]
          n241 = Multiply(x=8.0, y=w550) -> (x*y=w548:dbl)
          n242 = Replace Array Subset "Replace Array Subset"(array=w505, new element=w508, index=18) -> (w493:T1)
          n243 = Multiply(x=8.0, y=w563) -> (x*y=w561:dbl)
          n244 = Index Array "Index Array"(array=w493, index=30) -> (element=w498:T4)
          n245 = Unbundle By Name "Unbundle By Name"(w498) -> ("Instruct Data"=w504:i32, "Op Code"=w503:i32, "Flags"=w502:bool[], "Comments"=w501:string, "Time (s)"=w500:dbl)
          n246 = Add(x=w500, y=w495) -> (x+y=w499:dbl)
          "x+y 15" <- w499
          n247 = Bundle("Instruct Data"=w504, "Op Code"=w503, "Flags"=w502, "Comments"=w501, w499) -> (w496:T5)  [unwired: 1 in]
          n248 = Divide(x=w370, y=2.0) -> (x/y=w369:sgl)
          n249 = Replace Array Subset "Replace Array Subset"(array=w493, new element=w496, index=30) -> (w386:T1)
          n250 = Divide(x=w367, y=2.0) -> (x/y=w366:sgl)
          n251 = Index Array "Index Array"(array=w386, index=32) -> (element=w486:T4)
          n252 = Unbundle By Name "Unbundle By Name"(w486) -> ("Instruct Data"=w492:i32, "Op Code"=w491:i32, "Flags"=w490:bool[], "Comments"=w489:string, "Time (s)"=w488:dbl)
          n253 = Add(x=w488, y=w483) -> (x+y=w487:dbl)
          "x+y 16" <- w487
          n254 = Bundle("Instruct Data"=w492, "Op Code"=w491, "Flags"=w490, "Comments"=w489, w487) -> (w484:T5)  [unwired: 1 in]
          n255 = Divide(x=w364, y=2.0) -> (x/y=w363:sgl)
          n256 = Replace Array Subset "Replace Array Subset"(array=w386, new element=w484, index=32) -> (w385:T1)
          n257 = Divide(x=w373, y=2.0) -> (x/y=w372:dbl)
          n258 = Index Array "Index Array"(array=w385, index=34) -> (element=w475:T4)
          n259 = Unbundle By Name "Unbundle By Name"(w475) -> ("Instruct Data"=w481:i32, "Op Code"=w480:i32, "Flags"=w479:bool[], "Comments"=w478:string, "Time (s)"=w477:dbl)
          n260 = Add(x=w477, y=w472) -> (x+y=w476:dbl)
          "x+y 17" <- w476
          n261 = Bundle("Instruct Data"=w481, "Op Code"=w480, "Flags"=w479, "Comments"=w478, w476) -> (w473:T5)  [unwired: 1 in]
          n262 = Replace Array Subset "Replace Array Subset"(array=w385, new element=w473, index=34) -> (w384:T1)
          n263 = Index Array "Index Array"(array=w384, index=36) -> (element=w464:T4)
          n264 = Unbundle By Name "Unbundle By Name"(w464) -> ("Instruct Data"=w470:i32, "Op Code"=w469:i32, "Flags"=w468:bool[], "Comments"=w467:string, "Time (s)"=w466:dbl)
          n265 = Add(x=w466, y=w461) -> (x+y=w465:dbl)
          "x+y 18" <- w465
          n266 = Bundle("Instruct Data"=w470, "Op Code"=w469, "Flags"=w468, "Comments"=w467, w465) -> (w462:T5)  [unwired: 1 in]
          n267 = Replace Array Subset "Replace Array Subset"(array=w384, new element=w462, index=36) -> (w383:T1)
          n268 = Index Array "Index Array"(array=w383, index=38) -> (element=w453:T4)
          n269 = Unbundle By Name "Unbundle By Name"(w453) -> ("Instruct Data"=w459:i32, "Op Code"=w458:i32, "Flags"=w457:bool[], "Comments"=w456:string, "Time (s)"=w455:dbl)
          n270 = Add(x=w455, y=w450) -> (x+y=w454:dbl)
          "x+y 19" <- w454
          n271 = Bundle("Instruct Data"=w459, "Op Code"=w458, "Flags"=w457, "Comments"=w456, w454) -> (w451:T5)  [unwired: 1 in]
          n272 = Replace Array Subset "Replace Array Subset"(array=w383, new element=w451, index=38) -> (w382:T1)
          n273 = Index Array "Index Array"(array=w382, index=40) -> (element=w431:T4)
          n274 = Unbundle By Name "Unbundle By Name"(w431) -> ("Instruct Data"=w437:i32, "Op Code"=w436:i32, "Flags"=w435:bool[], "Comments"=w434:string, "Time (s)"=w433:dbl)
          n275 = Add(x=w433, y=w428) -> (x+y=w432:dbl)
          "x+y 21" <- w432
          n276 = Bundle("Instruct Data"=w437, "Op Code"=w436, "Flags"=w435, "Comments"=w434, w432) -> (w429:T5)  [unwired: 1 in]
          n277 = Replace Array Subset "Replace Array Subset"(array=w382, new element=w429, index=40) -> (w381:T1)
          n278 = Index Array "Index Array"(array=w381, index=42) -> (element=w442:T4)
          n279 = Unbundle By Name "Unbundle By Name"(w442) -> ("Instruct Data"=w448:i32, "Op Code"=w447:i32, "Flags"=w446:bool[], "Comments"=w445:string, "Time (s)"=w444:dbl)
          n280 = Add(x=w444, y=w439) -> (x+y=w443:dbl)
          "x+y 20" <- w443
          n281 = Bundle("Instruct Data"=w448, "Op Code"=w447, "Flags"=w446, "Comments"=w445, w443) -> (w440:T5)  [unwired: 1 in]
          n282 = Replace Array Subset "Replace Array Subset"(array=w381, new element=w440, index=42) -> (w380:T1)
          n283 = Index Array "Index Array"(array=w380, index=4) -> (element=w410:T4)
          n284 = Unbundle By Name "Unbundle By Name"(w410) -> ("Instruct Data"=w416:i32, "Op Code"=w415:i32, "Flags"=w414:bool[], "Comments"=w413:string, "Time (s)"=w412:dbl)
          n285 = Add(x=w412, y=w372) -> (x+y=w411:dbl)
          "x+y 23" <- w411
          n286 = Bundle("Instruct Data"=w416, "Op Code"=w415, "Flags"=w414, "Comments"=w413, w411) -> (w408:T5)  [unwired: 1 in]
          n287 = Replace Array Subset "Replace Array Subset"(array=w380, new element=w408, index=4) -> (w379:T1)
          n288 = Index Array "Index Array"(array=w379, index=20) -> (element=w420:T4)
          n289 = Unbundle By Name "Unbundle By Name"(w420) -> ("Instruct Data"=w426:i32, "Op Code"=w425:i32, "Flags"=w424:bool[], "Comments"=w423:string, "Time (s)"=w422:dbl)
          n290 = Add(x=w422, y=w363) -> (x+y=w421:dbl)
          "x+y 22" <- w421
          n291 = Bundle("Instruct Data"=w426, "Op Code"=w425, "Flags"=w424, "Comments"=w423, w421) -> (w418:T5)  [unwired: 1 in]
          n292 = Replace Array Subset "Replace Array Subset"(array=w379, new element=w418, index=20) -> (w378:T1)
          n293 = Index Array "Index Array"(array=w378, index=28) -> (element=w390:T4)
          n294 = Unbundle By Name "Unbundle By Name"(w390) -> ("Instruct Data"=w396:i32, "Op Code"=w395:i32, "Flags"=w394:bool[], "Comments"=w393:string, "Time (s)"=w392:dbl)
          n295 = Add(x=w392, y=w366) -> (x+y=w391:dbl)
          "x+y 25" <- w391
          n296 = Bundle("Instruct Data"=w396, "Op Code"=w395, "Flags"=w394, "Comments"=w393, w391) -> (w388:T5)  [unwired: 1 in]
          n297 = Replace Array Subset "Replace Array Subset"(array=w378, new element=w388, index=28) -> (w377:T1)
          n298 = Index Array "Index Array"(array=w377, index=44) -> (element=w400:T4)
          n299 = Unbundle By Name "Unbundle By Name"(w400) -> ("Instruct Data"=w406:i32, "Op Code"=w405:i32, "Flags"=w404:bool[], "Comments"=w403:string, "Time (s)"=w402:dbl)
          n300 = Add(x=w402, y=w369) -> (x+y=w401:dbl)
          "x+y 24" <- w401
          n301 = Bundle("Instruct Data"=w406, "Op Code"=w405, "Flags"=w404, "Comments"=w403, w401) -> (w398:T5)  [unwired: 1 in]
          n302 = Replace Array Subset "Replace Array Subset"(array=w377, new element=w398, index=44) -> (w376:T1)
          n303 = Index Array "Index Array"(array=w376, index=1) -> (element=w566:T4)
          n304 = Unbundle By Name "Unbundle By Name"(w566) -> ("Instruct Data"=w572:i32, "Op Code"=w571:i32, "Flags"=w570:bool[], "Comments"=w569:string, "Time (s)"=w568:dbl)
          n305 = Subtract(x=w568, y=w561) -> (x-y=w567:dbl)
          "x+y 5" <- w567
          n306 = Bundle("Instruct Data"=w572, "Op Code"=w571, "Flags"=w570, "Comments"=w569, w567) -> (w564:T5)  [unwired: 1 in]
          n307 = Replace Array Subset "Replace Array Subset"(array=w376, new element=w564, index=1) -> (w547:T1)
          n308 = Index Array "Index Array"(array=w547, index=25) -> (element=w553:T4)
          n309 = Unbundle By Name(w553) -> ("Instruct Data"=w559:i32, "Op Code"=w558:i32, "Flags"=w557:bool[], "Comments"=w556:string, "Time (s)"=w555:dbl)
          n310 = Subtract(x=w555, y=w548) -> (x-y=w554:dbl)
          "x+y 6" <- w554
          n311 = property on="Instructions" class="Arr (strict)"(error in=errorcluster {"status"=FALSE, "code"=0, "source"=""} ("error in (no error)"), "Number of Columns"=w543) -> (error out=w614:errorcluster)  [unwired: 1 in, 1 out]
          n312 = Bundle("Instruct Data"=w559, "Op Code"=w558, "Flags"=w557, "Comments"=w556, w554) -> (w551:T5)  [unwired: 1 in]
          n313 = global read "SpinCore_API_file_location.vi" "Path"() -> (w615:path)
          n314 = Replace Array Subset "Replace Array Subset"(array=w547, new element=w551, index=25) -> (w546:T1)
          "output array" <- w546
          n315 = call "pb_init.vi"("error in (no error)"=w614, "path in"=w615) -> ("error out"=w613:errorcluster, "path out"=w612:path)  [unwired: 8 in]
          n316 = call "pb_core_clock.vi"("error in (no error)"=w613, "clock_freq (MHz)"="clock_freq (MHz)", "path in"=w612) -> ("error out"=w629:errorcluster, "path out"=w630:path)  [unwired: 7 in]
          n317 = call "pb_start_programming.vi"("error in (no error)"=w629, "Device"=T3."Pulse Program", "path in"=w630) -> ("error out"=w636:errorcluster, "path out"=w640:path)  [unwired: 1 in, 6 out]
          n318 = for {
            tunnel: w546 -> [w703] mode=indexing
            shift-right: [w705] -> w638
            shift-left: w640 -> [w706]
            shift-right: [w702] -> w635
            shift-left: w636 -> [w704]
            n319 = call "pb_inst_pbonly.vi"("error in (no error)"=w704, "PB Instruction"=w703, "path in"=w706) -> ("error out"=w702:errorcluster, "path out"=w705:path)  [unwired: 2 in, 5 out]
          }
          n320 = call "pb_stop_programming.vi"("error in (no error)"=w635, "path in"=w638) -> ("error out"=w634:errorcluster, "path out"=w639:path)  [unwired: 1 in, 7 out]
          n321 = call "pb_close.vi"("error in (no error)"=w634, "path in"=w639) -> ("error out"=w627:errorcluster)  [unwired: 9 out]
          n322 = call "General Error Handler MOD.vi"("type of dialog (OK msg:1)"=DialogTypeEnum."continue or stop message", "error in (no error)"=w627) -> ("STOP?"=w631:bool, "error out"=w632:errorcluster)  [unwired: 12 out]
          n323 = case shown="False" w631 {
            tunnel: w632 -> [_ w701]
            frame False {
            }
            frame True {
              n324 = call <vilib>:"Clear Errors.vi"("error in (no error)"=w701) -> ()  [unwired: 1 in, 6 out]
            }
          }
        }
        frame #1 {
          n325 = Wait (ms)(milliseconds to wait=u32 1) -> ()  [unwired: 1 out]
        }
      }
    }
  }
  "Tau" <- w1
